vi "Write Time Entry File.vi"(7 "Task Names":string[](array[string]), 8 "error in (no error)":errorcluster, 9 "Project Names":string[](array[string]), 10 "Time Entries":T1, 11 "File Path":path) -> (0 "error out":errorcluster)   [LabVIEW 2024]
doc: "Writes a whole month file (a FULL REWRITE) from the given time entries, sorted by Start Time, with the [_Meta] section and the Project Name and Task Name labels. Project Names and Task Names run parallel to Time Entries. Timestamps are written as ISO 8601 UTC; an End Time of 0 is written as an empty string (a running entry).\n\nGenerated by: Claude"
uses:
  Utilities/Time Management/Time Management.lvlib
  Rows/Time Entry.ctl
  Rows/Time Entry List.ctl
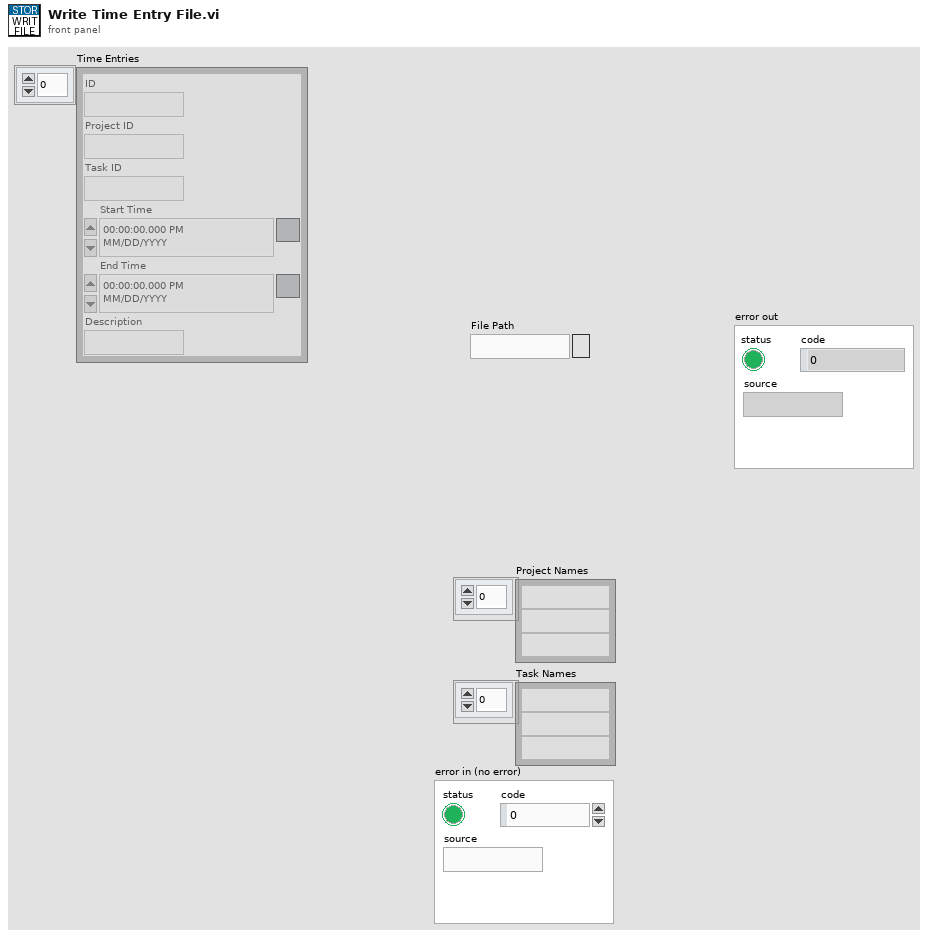
[diagram p1: front panel]
types:
  T1 = typedef "Time Entry List.ctl" = T2[]
  T2 = typedef "Time Entry.ctl" = cluster{"ID":string, "Project ID":string, "Task ID":string, "Start Time":timestamp, "End Time":timestamp, "Description":string}
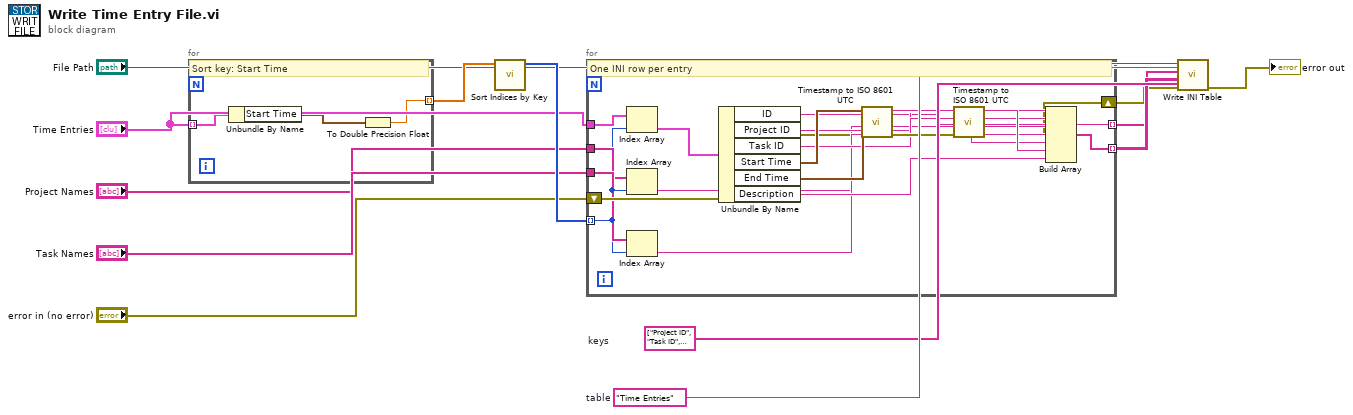
[diagram p0: block diagram]
diagram:
  w12 = "Time Entries"  # table
  w11 = string[] ["Project ID", "Task ID", "Project Name", "Task Name", "Start Time", "End Time", "Description"]  # keys
  n1 = for {
    tunnel: "Time Entries" -> [w14] mode=indexing
    tunnel: [w16] -> w6 mode=indexing
    # "Sort key: Start Time"
    n2 = Unbundle By Name(w14) -> ("Start Time"=w15:timestamp)
    n3 = To Double Precision Float(number=w15) -> (double precision float=w16:dbl)
  }
  n4 = call "Sort Indices by Key.vi"("Keys"=w6) -> ("Sorted Indices"=w7:i32[])  [unwired: 9 in, 1 out]
  n5 = for {
    tunnel: "Time Entries" -> [w18]
    tunnel: "Project Names" -> [w19]
    tunnel: "Task Names" -> [w20]
    shift-right: [w22] -> w8
    shift-left: "error in (no error)" -> [w21]
    tunnel: w7 -> [w17] mode=indexing
    tunnel: [w26] -> w9 mode=indexing
    tunnel: [w35] -> w10 mode=indexing
    # "One INI row per entry"
    n6 = Index Array(array=w18, index=w17) -> (element=w23:T2)
    n7 = Index Array(array=w19, index=w17) -> (element=w24:string)
    n8 = Index Array(array=w20, index=w17) -> (element=w25:string)
    n9 = Unbundle By Name(w23) -> ("ID"=w26:string, "Project ID"=w27:string, "Task ID"=w28:string, "Start Time"=w29:timestamp, "End Time"=w30:timestamp, "Description"=w31:string)
    n10 = call "Timestamp to ISO 8601 UTC.vi"("error in (no error)"=w21, "Timestamp"=w29) -> ("error out"=w33:errorcluster, "ISO 8601 UTC"=w32:string)  [unwired: 8 in]
    n11 = call "Timestamp to ISO 8601 UTC.vi"("error in (no error)"=w33, "Timestamp"=w30) -> ("error out"=w22:errorcluster, "ISO 8601 UTC"=w34:string)  [unwired: 8 in]
    n12 = Build Array(w27, w28, w24, w25, w32, w34, w31) -> (w35:string[])
  }
  n13 = call "Write INI Table.vi"("Keys"=w11, "Table Name"=w12, "error in (no error)"=w8, "Values"=w10, "Section Names"=w9, "File Path"="File Path") -> ("error out"=→"error out":errorcluster)  [unwired: 5 in]
